vi "Get Exposure Time Representation.vi"(8 "error in (no error)":errorcluster, 11 "Camera in":refnum<class "Camera.lvclass">) -> (0 "error out":errorcluster, 2 "Representation":T1, 3 "Camera":refnum<class "Camera.lvclass">)   [LabVIEW 2020, in "Camera.lvclass"]
uses:
  Camera.lvclass
  Representation.ctl
  Camera.lvclass/Camera.ctl
  bin/gindustrialcam_32-1.dll
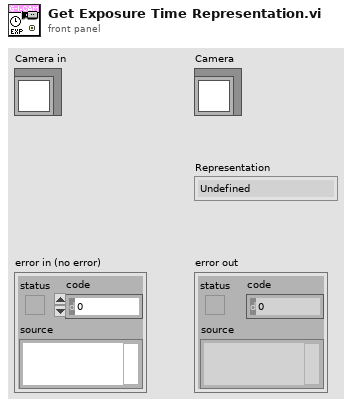
[diagram p1: front panel]
types:
  T1 = typedef "Camera.lvclass/Representation.ctl" = enum8{"Undefined", "Linear", "Logarithmic", "Boolean", "Pure Number", "Hex Number", "IP Address", "MAC Address"}
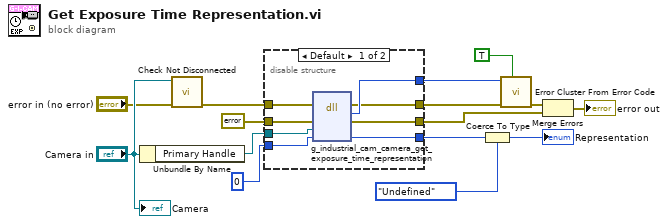
[diagram p0: block diagram]
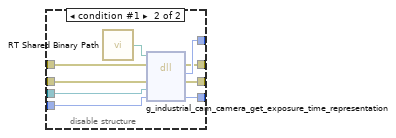
[diagram p2: hidden frame]
diagram:
  n1 = Unbundle By Name("Camera in") -> ("Primary Handle"=w11:refnum<data-value>)
  n2 = call "Check Not Disconnected.vi"("error in (no error)"="error in (no error)", "Camera in"="Camera in") -> ("error out"=w12:errorcluster)  [unwired: 9 in]
  n3 = disable-structure shown="Default" {
    disable-tunnel: w12 -> [w23 w32]
    disable-tunnel: w11 -> [w22 w31]
    disable-tunnel: errorcluster {"status"=FALSE, "code"=0, "source"=""} ("error constant") -> [w21 w30]
    disable-tunnel: [w20 w29] -> w8
    disable-tunnel: [w19 w28] -> w6
    disable-tunnel: [w18 w27] -> w5
    disable-tunnel: [w17 w26] -> w4
    disable-tunnel: u8 0 ("representation") -> [w16 w25]
    frame condition #0 (active) {
      n4 = dll-call lib="C:/serenial/lib/g-industrial-camera/LabVIEW/g_industrial_cam/bin/gindustrialcam_*-1.*" fn="g_industrial_cam_camera_get_exposure_time_representation"(error in=w23, "err"=w21, "edvr"=w22, "representation"=w16) -> (error out=w18:errorcluster, "Mg_Error"=w19:i32, "err"=w20:errorcluster, "representation"=w17:u8)  [unwired: 3 in, 1 out]
    }
    frame condition #1 {
      n5 = call "RT Shared Binary Path.vi"() -> ("Path"=w24:path)
      n6 = dll-call lib="C:/serenial/lib/g-industrial-camera/LabVIEW/g_industrial_cam/bin/gindustrialcam_*-1.*" fn="g_industrial_cam_camera_get_exposure_time_representation"(path in=w24, error in=w32, "err"=w30, "edvr"=w31, "representation"=w25) -> (error out=w27:errorcluster, "Mg_Error"=w28:i32, "err"=w29:errorcluster, "representation"=w26:u8)  [unwired: 2 in, 1 out]
    }
  }
  n7 = Coerce To Type(0:w4, 1:Representation."Undefined" ("Representation")) -> (2:→"Representation":T1)
  n8 = call <vilib>:"Error Cluster From Error Code.vi"("show call chain? (False)"=TRUE, "error in (no error)"=w5, "error code (0)"=w6) -> ("error out"=w7:errorcluster)  [unwired: 6 in]
  n9 = Merge Errors(w7, w8) -> (→"error out":errorcluster)
  "Camera" <- "Camera in"
